vi "Iceoryx Channel Errors Core.vi"(8 "error in (no error)":errorcluster, 10 "String to Append":string, 11 "Error":T1) -> (0 "error out":errorcluster)   [LabVIEW 2021, in "CIF_Iceoryx_Chn.lvclass"]
uses:
  CIF_Iceoryx_Chn.lvclass
  Typedef/Iceoryx Channel Error.ctl
  <vilib>/CIF Foundation/CIF Utilities/Errors/Errors_CIF_U.lvlib
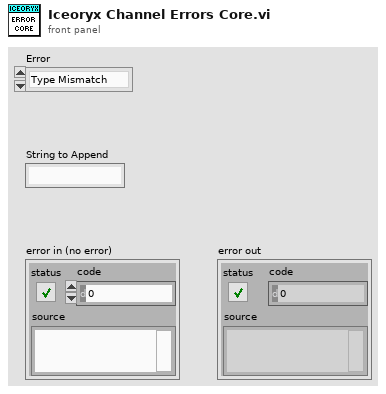
[diagram p1: front panel]
types:
  T1 = typedef "CIF_Iceoryx_Chn.lvclass/Iceoryx Channel Error.ctl" = enum16{"Type Mismatch", "Name Mismatch", "Override Required"}
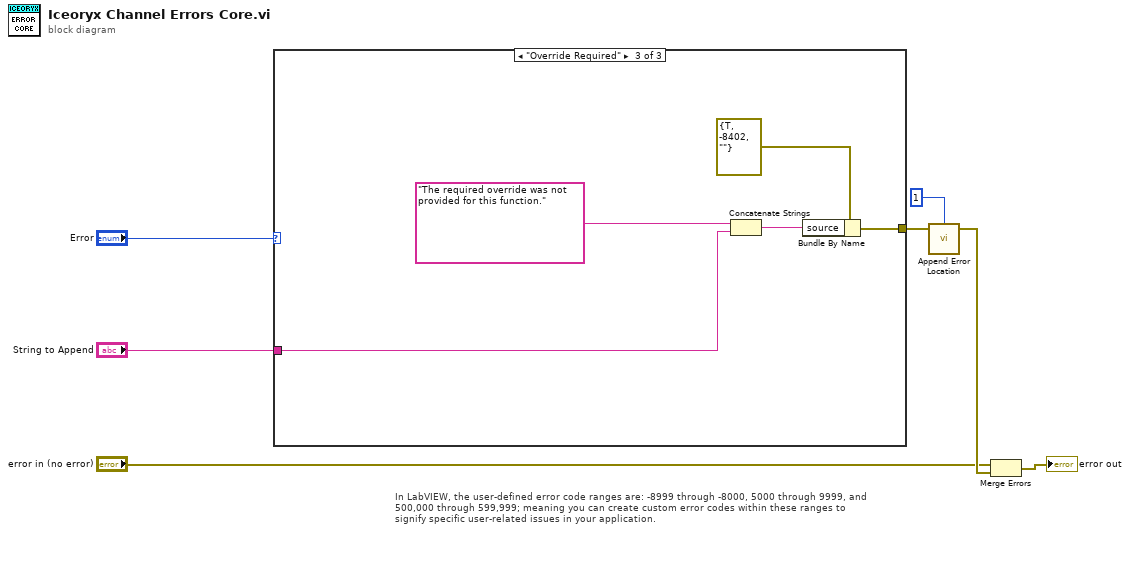
[diagram p0: block diagram]
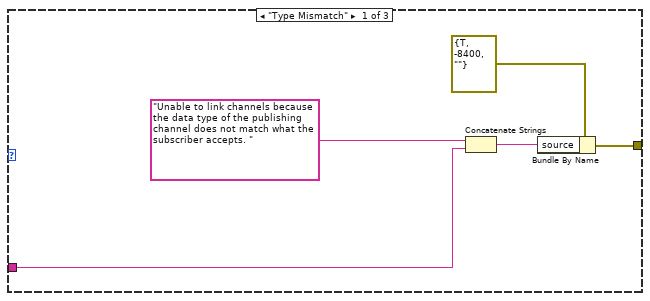
[diagram p2: hidden frame]
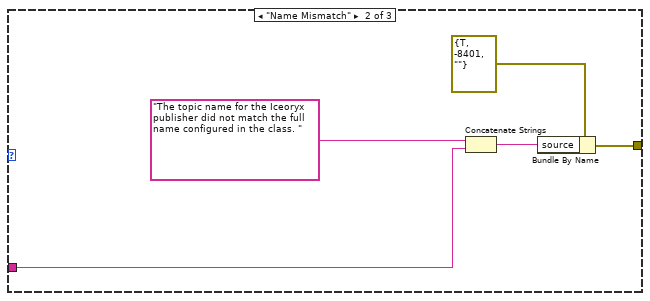
[diagram p3: hidden frame]
diagram:
  # "In LabVIEW, the user-defined error code ranges are: -8999 through -8000, 5000 through 9999, and 500,000 through 599,999; meaning you can create custom error codes within these ranges to signify specific user-related issues in your application."
  n1 = case shown="\"Override Required\"" "Error" {
    tunnel: "String to Append" -> [w8 w13 w18]
    tunnel: [w11 w16 w21] -> w6
    frame "Type Mismatch" {
      n2 = Concatenate Strings("Unable to link channels because the data type of the publishing channel does not match what the subscriber accepts. " ("source"), w8) -> (w9:string)
      n3 = Bundle By Name(cluster=errorcluster {"status"=TRUE, "code"=-8400, "source"=""} ("Invalid ID"), "source"=w9) -> (w11:errorcluster)
    }
    frame "Name Mismatch" {
      n4 = Concatenate Strings("The topic name for the Iceoryx publisher did not match the full name configured in the class. " ("source"), w13) -> (w14:string)
      n5 = Bundle By Name(cluster=errorcluster {"status"=TRUE, "code"=-8401, "source"=""} ("Invalid ID"), "source"=w14) -> (w16:errorcluster)
    }
    frame "Override Required" {
      n6 = Concatenate Strings("The required override was not provided for this function." ("source"), w18) -> (w19:string)
      n7 = Bundle By Name(cluster=errorcluster {"status"=TRUE, "code"=-8402, "source"=""} ("Invalid ID"), "source"=w19) -> (w21:errorcluster)
    }
  }
  n8 = call <vilib>:"Append Error Location.vi"("error in (no error)"=w6, "Chain Depth"=1) -> ("error out"=w7:errorcluster)  [unwired: 3 in]
  n9 = Merge Errors("error in (no error)", w7) -> (→"error out":errorcluster)
